vi "Read All Stderr.vi"(6 "Per Read Size":i32=1024 max=30000, 8 "Error In":errorcluster, 10 "Total Read Size":i32=1024, 11 "Channel In":refnum<class "Channel.lvclass">) -> (0 "Error Out":errorcluster, 1 "Timed Out?":bool, 2 "Data":u8[](array[numeric]), 3 "Channel Out":refnum<class "Channel.lvclass">)   [LabVIEW 2018, in "Toolkit.lvlib" / "Channel.lvclass"]
doc: "Reads binary data from the STDERR stream of a SSH channel represented by this Channel object in chunks, or blocks, until the total read size is reached. This VI should be used if the <B>Total Read Size</B> is greater than 30KB because of a hard-coded per-read maximum of 30KB defined in the libssh2 shared library."
uses:
  Channel.lvclass
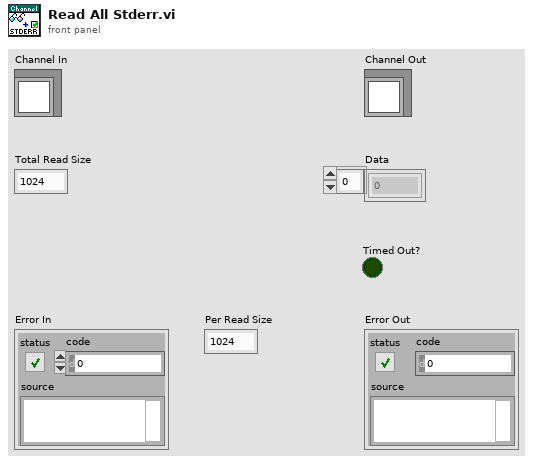
[diagram p1: front panel]
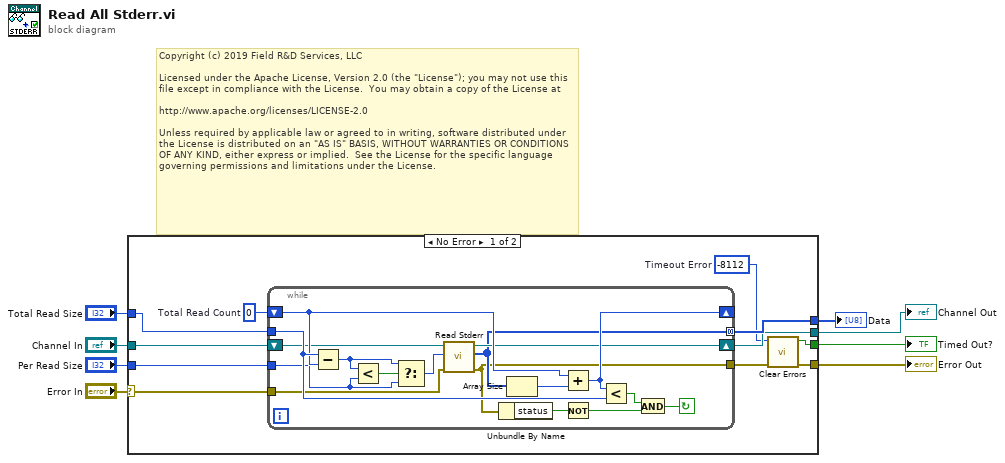
[diagram p0: block diagram]
diagram:
  # "Copyright (c) 2019 Field R&D Services, LLC\n\nLicensed under the Apache License, Version 2.0 (the \"License\"); you may not use this file except in compliance with the License.  You may obtain a copy of the License at\n\nhttp://www.apache.org/licenses/LICENSE-2.0\n\nUnless required by applicable law or agreed to in writing, software distributed under the License is distributed on an \"AS IS\" BASIS, WITHOUT WARRANTIES OR CONDITIONS OF ANY KIND, either express or implied.  See the License for the specific language governing permissions and limitations under the License."
  n1 = case shown="No Error" "Error In" {
    selector: "Error In" -> [w13 w37]
    tunnel: "Total Read Size" -> [w18 _]
    tunnel: "Per Read Size" -> [w17 _]
    tunnel: "Channel In" -> [w16 w38]
    tunnel: [w15 _] -> w5
    tunnel: [w14 w38] -> w4
    tunnel: [w11 w37] -> w3
    tunnel: [w9 _] -> w1
    frame No Error {
      w10 = -8112  # Timeout Error
      w19 = 0  # Total Read Count
      n2 = while {
        shift-right: [w29] -> w14
        shift-left: w16 -> [w26]
        tunnel: [w28] -> w15 mode=concatenating
        shift-right: [w35] -> _
        shift-left: w19 -> [w33]
        tunnel: w18 -> [w34]
        tunnel: w17 -> [w30]
        tunnel: w13 -> [w25]
        tunnel: [w22] -> w12
        stop <- w20 continue-if-true
        n3 = Subtract(x=w34, y=w33) -> (x-y=w31:i32)
        n4 = Less?(x=w31, y=w30) -> (x < y?=w32:bool)
        n5 = Select(t=w31, s=w32, f=w30) -> (s? t:f=w27:i32)
        n6 = call "Read Stderr.vi"("Error In"=w25, "Max Data Length"=w27, "Channel In"=w26) -> ("Error Out"=w22:errorcluster, "Data"=w28:u8[], "Channel Out"=w29:refnum<class "Channel.lvclass">)  [unwired: 6 in]
        n7 = Unbundle By Name(w22) -> ("status"=w21:bool)
        n8 = Array Size(array=w28) -> (size(s)=w36:i32)
        n9 = Add(x=w33, y=w36) -> (x+y=w35:i32)
        n10 = Not(x=w21) -> (.not. x?=w24:bool)
        n11 = Less?(x=w35, y=w34) -> (x < y?=w23:bool)
        n12 = And(x=w23, y=w24) -> (x .and. y?=w20:bool)
      }
      n13 = call <vilib>:"Clear Errors.vi"("error in (no error)"=w12, "specific error code to clear (0: all)"=w10) -> ("error out"=w11:errorcluster, "specific error cleared?"=w9:bool)  [unwired: 4 in]
    }
    frame Error {
    }
  }
  "Data" <- w5
  "Channel Out" <- w4
  "Error Out" <- w3
  "Timed Out?" <- w1
